vi "RemoteVI Get Panel Geometry.vi"(0 "VI":refnum<vi>, 11 "error in":errorcluster) -> (4 "geo":T1, 6 "hWnd":u64, 8 "origin":cluster{"x":i32, "y":i32}, 15 "error out":errorcluster)   [LabVIEW 2020, in "RemoteVI.lvlib"]
doc: "Reads where the front panel window of VI is on screen, for RemoteVI Translate Input.vi and the overlay. The browser shows the FRAME - the whole window below its title bar, i.e. its client area with LabVIEW's menu bar, toolbar, panel and scrollbars (RemoteVI Frame Rect.vi) - so the coordinates a client sends are frame coordinates: geo.panelX/panelY = the screen position of the frame's top-left corner (the point browser coordinates are relative to; the name is historical - it was the panel origin while only the panel was streamed), geo.clientX/clientY = the screen position of the window's client-area origin (the negative of user32 ScreenToClient applied to the screen point 0,0). Both are the same point today, because the frame is the client area. origin = where the panel area (Front Panel Window:Panel Bounds left/top) starts inside the frame - below the menu bar and the toolbar - sent to the clients as the text message origin x y (docs\\protocol.md 3.3). Also returns the window handle (Front Panel Window:OS Window, sign-extended I32 to I64 to U64). A VI Server call: the server loop calls it before its first iteration and then every 500 ms while no popup is open. An incoming error skips the work."
uses:
  RemoteVI.lvlib
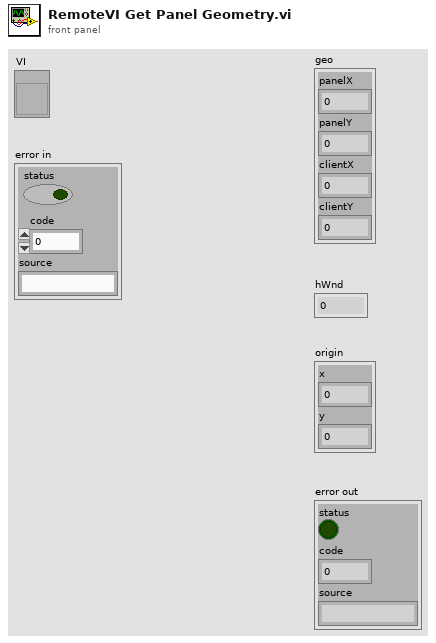
[diagram p1: front panel]
types:
  T1 = cluster{"panelX":i32, "panelY":i32, "clientX":i32, "clientY":i32}
  T2 = typedef "LVRectTypeDef.ctl" = cluster{"left":i16, "top":i16, "right":i16, "bottom":i16}
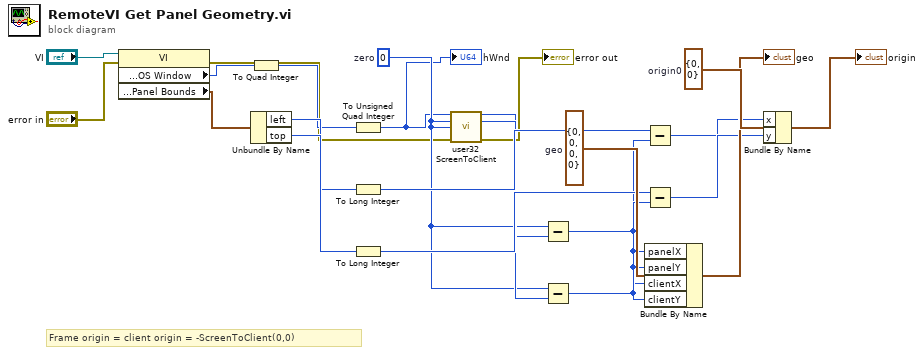
[diagram p0: block diagram]
diagram:
  w22 = cluster{"x":i32, "y":i32} {"x"=0, "y"=0}  # origin0
  w20 = T1 {"panelX"=0, "panelY"=0, "clientX"=0, "clientY"=0}  # geo
  w8 = 0  # zero
  # "Frame origin = client origin = -ScreenToClient(0,0)"
  n1 = property class="VI"(reference="VI", error in="error in") -> (error out=w3:errorcluster, "Front Panel Window:OS Window"=w4:i32, "Front Panel Window:Panel Bounds"=w5:T2)  [unwired: 1 out]
  n2 = To Quad Integer(1:w4) -> (0:w6:i64)
  n3 = Unbundle By Name(w5) -> ("left"=w14:i16, "top"=w15:i16)
  n4 = To Unsigned Quad Integer(1:w6) -> (0:w7:u64)
  "hWnd" <- w7
  n5 = To Long Integer(number=w14) -> (32bit integer=w16:i32)
  n6 = To Long Integer(number=w15) -> (32bit integer=w17:i32)
  n7 = call "user32 ScreenToClient.vi"("hWnd"=w7, "Screen X"=w8, "Screen Y"=w8, "error in (no error)"=w3) -> ("Client X"=w9:i32, "Client Y"=w10:i32, "error out"=→"error out":errorcluster)  [unwired: 8 in, 1 out]
  n8 = Subtract(x=w8, y=w9) -> (x-y=w12:i32)
  n9 = Subtract(x=w8, y=w10) -> (x-y=w13:i32)
  n10 = Subtract(x=w16, y=w12) -> (x-y=w18:i32)
  n11 = Subtract(x=w17, y=w13) -> (x-y=w19:i32)
  n12 = Bundle By Name(cluster=w20, "panelX"=w12, "panelY"=w13, "clientX"=w12, "clientY"=w13) -> (→"geo":T1)
  n13 = Bundle By Name(cluster=w22, "x"=w18, "y"=w19) -> (→"origin":cluster{"x":i32, "y":i32})
